vi "FRC Append Project Extension.vi"(8 "error in (no error)":errorcluster, 11 "project name":string) -> (0 "error out":errorcluster, 3 "project name out":string)   [LabVIEW 2027]
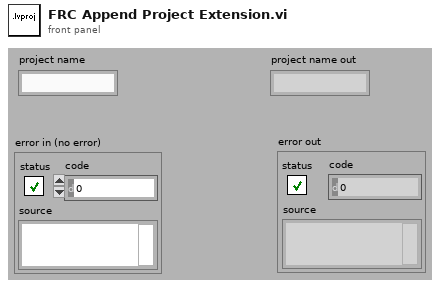
[diagram p1: front panel]
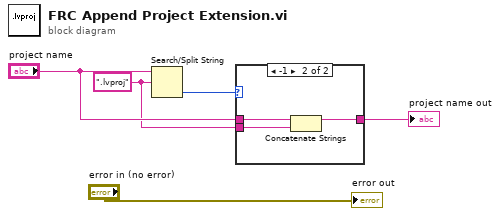
[diagram p0: block diagram]
diagram:
  w2 = ".lvproj" ("search string/char (-)")
  n1 = Search/Split String(string="project name", search string/char (-)=w2) -> (offset of match=w5:i32)  [unwired: 1 in, 2 out]
  n2 = case shown="-1" w5 {
    tunnel: [w6 w7] -> w3
    tunnel: "project name" -> [w6 w9]
    tunnel: w2 -> [_ w8]
    frame Default {
    }
    frame -1 {
      n3 = Concatenate Strings(w9, w8) -> (w7:string)
    }
  }
  "project name out" <- w3
  "error out" <- "error in (no error)"
